vi "Calculate Cascade FeedForward.vi"(11 "Setpoint":dbl) -> (3 "Arbitrary Feedforward":dbl)   [LabVIEW 2023]
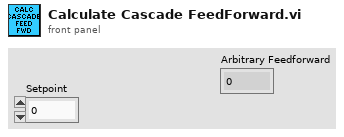
[diagram p1: front panel]
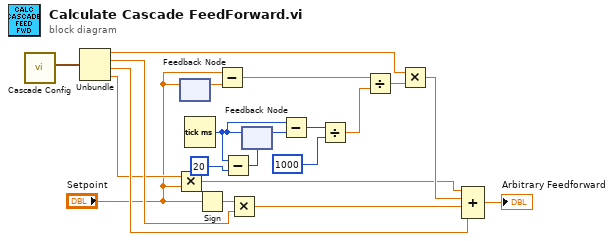
[diagram p0: block diagram]
diagram:
  n1 = call "Cascade Config.vi"() -> ("FeedForward Constants Out"=w4:cluster{"kA":dbl, "kS":dbl, "kG":dbl, "kV":dbl})  [unwired: 10 in, 1 out]
  n2 = Unbundle(w4) -> ("kA"=w10:dbl, "kS"=w9:dbl, "kG"=w8:dbl, "kV"=w7:dbl)
  n3 = Multiply(x=w7, y="Setpoint") -> (x*y=w5:dbl)
  n4 = feedback #1() -> (w19:dbl)  [unwired: 1 in]
  n5 = feedback-in #1("Setpoint") -> ()
  n6 = Tick Count (ms)() -> (millisecond timer value=w3:u32)
  n7 = Sign(1:"Setpoint") -> (0:w21:dbl)
  n8 = Subtract(x="Setpoint", y=w19) -> (x-y=w18:dbl)
  n9 = Subtract(x=w3, y=u32 20) -> (x-y=w1:u32)
  n10 = Multiply(x=w21, y=w9) -> (x*y=w20:dbl)
  n11 = feedback #2(w1) -> (w17:u32)
  n12 = feedback-in #2(w3) -> ()
  n13 = Subtract(x=w3, y=w17) -> (x-y=w16:u32)
  n14 = Divide(x=w16, y=u32 1000) -> (x/y=w14:dbl)
  n15 = Divide(x=w18, y=w14) -> (x/y=w13:dbl)
  n16 = Multiply(x=w10, y=w13) -> (x*y=w12:dbl)
  n17 = Compound Arithmetic op=ADD(w5, w12, w20, w8) -> (→"Arbitrary Feedforward":dbl)
